vi "KYFG Buffer Get Ptr.vi"(8 "error in (no error)":errorcluster, 10 "frame":u32, 11 "buffHandle":u32) -> (0 "error out":errorcluster, 3 "buffer data":u64)   [LabVIEW 2023, in "KYFGLib_lv.lvlib"]
doc: "KYFG_API void* KYFG_BufferGetPtr(BUFFHANDLE buffHandle , unsigned int frame);"
uses:
  KYFGLib_lv.lvlib
  KYFGLib.dll
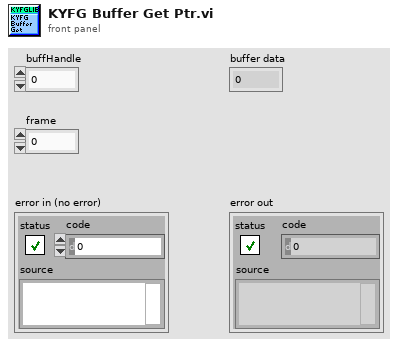
[diagram p1: front panel]
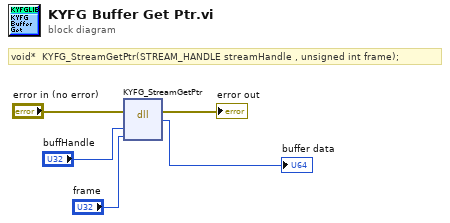
[diagram p0: block diagram]
diagram:
  # "void*\t\tKYFG_StreamGetPtr(STREAM_HANDLE streamHandle , unsigned int frame);"
  n1 = dll-call lib="KYFGLib.dll" fn="KYFG_StreamGetPtr"(error in="error in (no error)", "streamHandle"="buffHandle", "frame"="frame") -> (error out=→"error out":errorcluster, "return type"=→"buffer data":u64)  [unwired: 4 in, 1 out]
